vi "OwnFile20261012_Native_GetTerminalTypeDescriptor.vi"() -> ()   [LabVIEW 2024]
panel:
  out "error out":errorcluster caption="错误输出"
  out "type_string":i16[](array[numeric])
  in  "terminal_id":u32
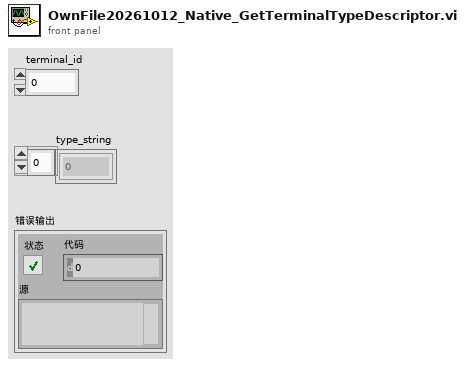
[diagram p1: front panel]
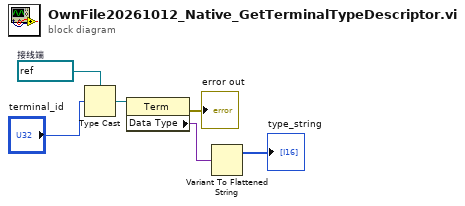
[diagram p0: block diagram]
diagram:
  w5 = refnum<vi> refnum  # 接线端
  n1 = Type Cast ("强制类型转换")(type=w5, x="terminal_id") -> (*(type *) &x=w4:refnum<vi>)
  n2 = property on="属性节点" class="Term"(reference=w4) -> (error out=→"error out":errorcluster, "Data Type"=w3:variant)  [unwired: 1 in, 1 out]
  n3 = Variant To Flattened String ("变体至平化字符串转换")(Variant=w3) -> (1:→"type_string":i16[])  [unwired: 1 out]
